vi "VIH ProjFile - Group Rule - Replace Obsolete Master JS Files.vi"(9 "Master Rule (F)":bool, 11 "Group Rule":T1) -> (1 "changed":bool, 3 "Group Rule out":T1)   [LabVIEW 2014]
doc: "::: VI Helpeks :::\nCopyright (c) 2000-2026 Konstantin Shifershteyn. All rights reserved."
uses:
  _VIH HelpGen.llb/VIH HelpGen Typedef - Cluster - Group Rule.ctl
  _VIH HelpGen.llb/VIH HelpGen Typedef - Enum - Default,Enable,Disable.ctl
  _VIH HelpGen.llb/VIH HelpGen Typedef - Cluster - Group Rule - Source Paths.ctl
  _VIH HelpGen.llb/VIH HelpGen Typedef - Cluster - Group Rule - Target Paths.ctl
  _VIH HelpGen.llb/VIH HelpGen Typedef - Enum - Description Mode.ctl
  _VIH HelpGen.llb/VIH HelpGen Typedef - Cluster - Control Rule.ctl
  _VIH HelpGen.llb/VIH HelpGen Typedef - Cluster - Enum Value Info.ctl
  _VIH HelpGen.llb/VIH HelpGen Typedef - Cluster - Group Rule - Flags.ctl
panel:
  # "VI Helpeks\nCopyright (c) 2012-2026 Konstantin Shifershteyn"
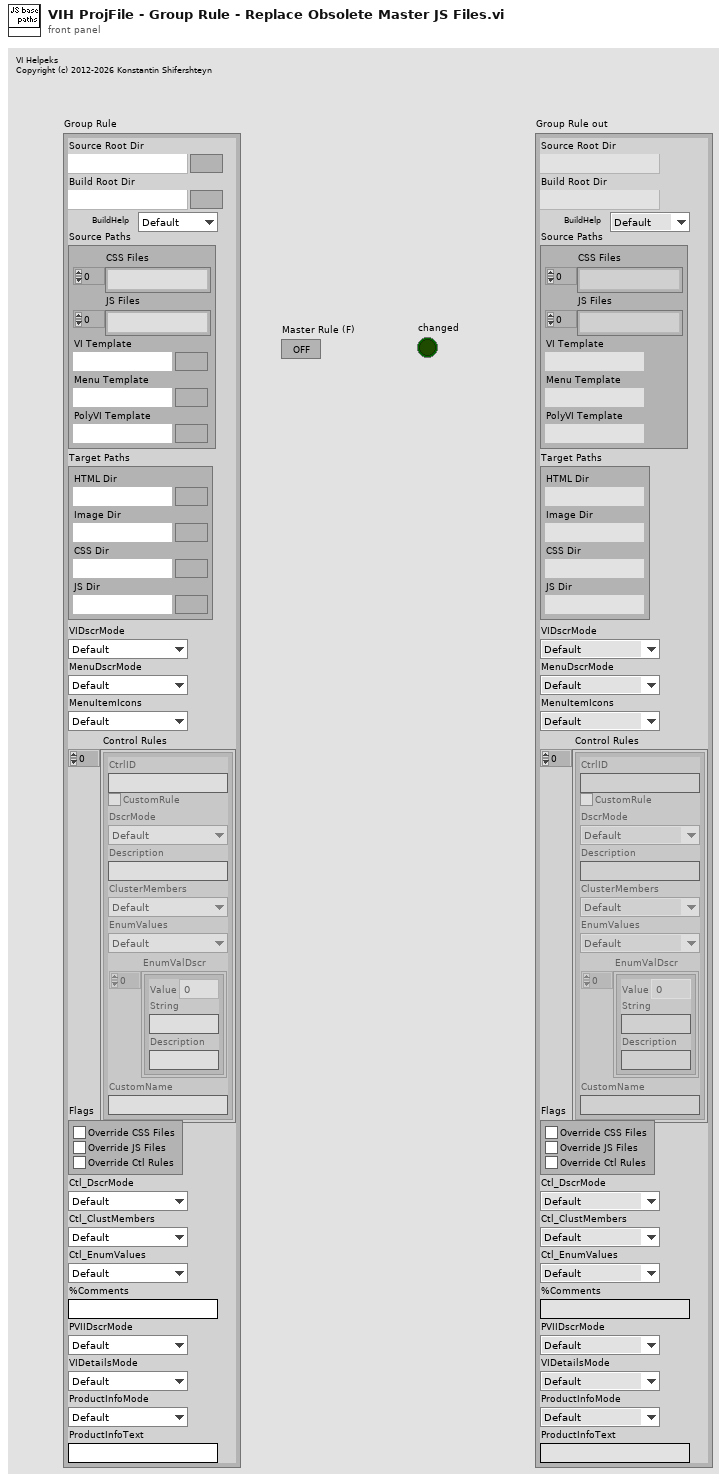
[diagram p1: front panel]
types:
  T1 = typedef "VIH HelpGen Typedef - Cluster - Group Rule.ctl" = cluster{"Source Root Dir":path, "Build Root Dir":path, "BuildHelp":T2, "Source Paths":T3, "Target Paths":T4, "VIDscrMode":T5, "MenuDscrMode":T5, "MenuItemIcons":T2, "Control Rules":T6[], "Flags":T8, "Ctl_DscrMode":T5, "Ctl_ClustMembers":T2, "Ctl_EnumValues":T2, "%Comments":string, "PVIIDscrMode":T5, "VIDetailsMode":T5, "ProductInfoMode":T2, "ProductInfoText":string}
  T2 = typedef "VIH HelpGen Typedef - Enum - Default,Enable,Disable.ctl" = enum16{"Default", "Enable", "Disable"}
  T3 = typedef "VIH HelpGen Typedef - Cluster - Group Rule - Source Paths.ctl" = cluster{"CSS Files":path[], "JS Files":path[], "VI Template":path, "Menu Template":path, "PolyVI Template":path}
  T4 = typedef "VIH HelpGen Typedef - Cluster - Group Rule - Target Paths.ctl" = cluster{"HTML Dir":path, "Image Dir":path, "CSS Dir":path, "JS Dir":path}
  T5 = typedef "VIH HelpGen Typedef - Enum - Description Mode.ctl" = enum16{"Default", "Description", "Description1", "Description2", "Custom", "None"}
  T6 = typedef "VIH HelpGen Typedef - Cluster - Control Rule.ctl" = cluster{"CtrlID":string, "CustomRule":bool, "DscrMode":T5, "Description":string, "ClusterMembers":T2, "EnumValues":T2, "EnumValDscr":T7[], "CustomName":string}
  T7 = typedef "VIH HelpGen Typedef - Cluster - Enum Value Info.ctl" = cluster{"Value":ext, "String":string, "Description":string}
  T8 = typedef "VIH HelpGen Typedef - Cluster - Group Rule - Flags.ctl" = cluster{"Override CSS Files":bool, "Override JS Files":bool, "Override Ctl Rules":bool}
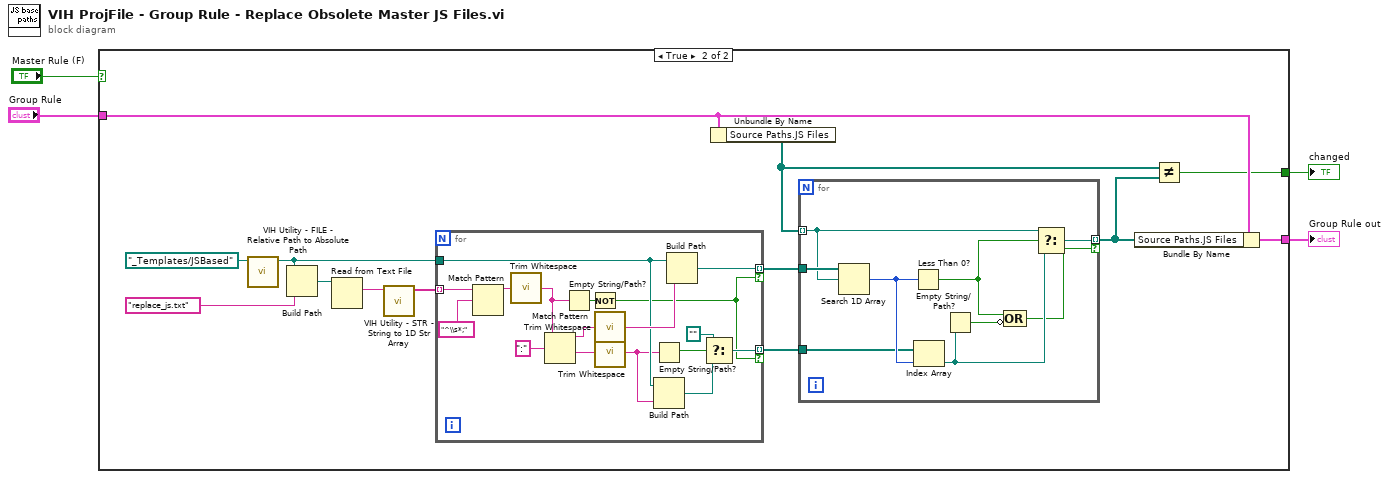
[diagram p0: block diagram]
diagram:
  n1 = case shown="True" "Master Rule (F)" {
    tunnel: "Group Rule" -> [w5 w18]
    tunnel: [w5 w17] -> w3
    tunnel: [_ w16] -> w1
    frame False {
    }
    frame True {
      n2 = call "VIH Utility - FILE - Relative Path to Absolute Path.vi"("Path"=path "_Templates/JSBased") -> ("Path out"=w13:path)  [unwired: 9 in, 1 out]
      n3 = Build Path(base path=w13, name or relative path="replace_js.txt") -> (appended path=w10:path)
      n4 = Read from Text File(file (use dialog)=w10) -> (text=w11:string)  [unwired: 3 in, 3 out]
      n5 = call "VIH Utility - STR - String to 1D Str Array.vi"("String in"=w11) -> ("Array out"=w12:string[])  [unwired: 6 in]
      n6 = for {
        tunnel: w12 -> [w35] mode=indexing
        tunnel: w13 -> [w28]
        tunnel: [w29] -> w7 mode=indexing if=w19
        tunnel: [w24] -> w6 mode=indexing if=w19
        n7 = Match Pattern(string=w35, regular expression="^\\s*;") -> (before substring=w22:string)  [unwired: 1 in, 3 out]
        n8 = call <vilib>:"Trim Whitespace.vi"("string"=w22) -> ("trimmed string"=w21:string)  [unwired: 1 in]
        n9 = Match Pattern(string=w21, regular expression=":") -> (before substring=w32:string, after substring=w31:string)  [unwired: 1 in, 2 out]
        n10 = Empty String/Path?(string/path=w21) -> (empty?=w20:bool)
        n11 = Not(x=w20) -> (.not. x?=w19:bool)
        n12 = call <vilib>:"Trim Whitespace.vi"("string"=w32) -> ("trimmed string"=w30:string)  [unwired: 1 in]
        n13 = call <vilib>:"Trim Whitespace.vi"("string"=w31) -> ("trimmed string"=w27:string)  [unwired: 1 in]
        n14 = Empty String/Path?(string/path=w27) -> (empty?=w26:bool)
        n15 = Build Path(base path=w28, name or relative path=w27) -> (appended path=w25:path)
        n16 = Build Path(base path=w28, name or relative path=w30) -> (appended path=w29:path)
        n17 = Select(t=path "", s=w26, f=w25) -> (s? t:f=w24:path)
      }
      n18 = Unbundle By Name(w18) -> ("Source Paths.JS Files"=w15:path[])
      n19 = for {
        tunnel: w15 -> [w42] mode=indexing
        tunnel: w7 -> [w44]
        tunnel: [w43] -> w14 mode=indexing if=w36
        tunnel: w6 -> [w40]
        n20 = Search 1D Array(1D array=w44, element=w42) -> (index of element=w41:i32)  [unwired: 1 in]
        n21 = Less Than 0?(x=w41) -> (x < 0?=w39:bool)
        n22 = Index Array(array=w40, index=w41) -> (element=w38:path)
        n23 = Empty String/Path?(string/path=w38) -> (empty?=w37:bool)
        n24 = Compound Arithmetic op=OR(w39, invert w37) -> (w36:bool)
        n25 = Select(t=w42, s=w39, f=w38) -> (s? t:f=w43:path)
      }
      n26 = Bundle By Name(cluster=w18, "Source Paths.JS Files"=w14) -> (w17:T1)
      n27 = Not Equal?(x=w15, y=w14) -> (x != y?=w16:bool)
    }
  }
  "Group Rule out" <- w3
  "changed" <- w1
